vi "Washing Machine.vi"() -> ()   [LabVIEW 2026]
doc: "Timed cyclic state machine for a washing machine: Soak, Wash, Rinse, Spin."
panel:
  out "History":enum16{"Soak", "Wash", "Rinse", "Spin"}[](array[ring])
  out "Cycles":i32
  out "Final Tick":i32
  out "Final State":enum16{"Soak", "Wash", "Rinse", "Spin"}(ring)
  in  "Max Cycles":i32=2
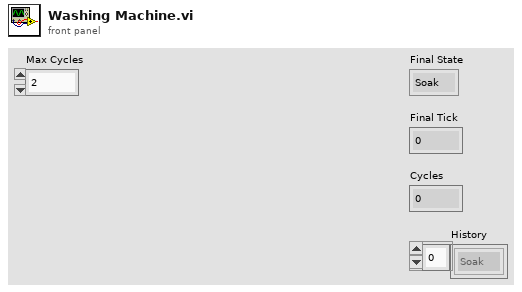
[diagram p1: front panel]
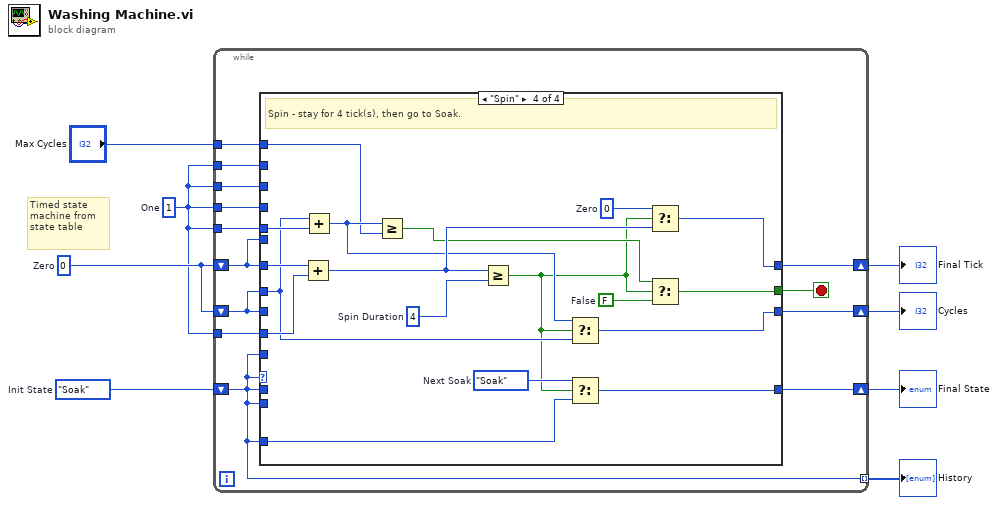
[diagram p0: block diagram]
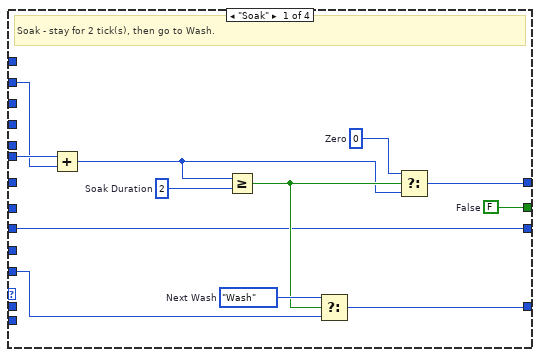
[diagram p2: hidden frame]
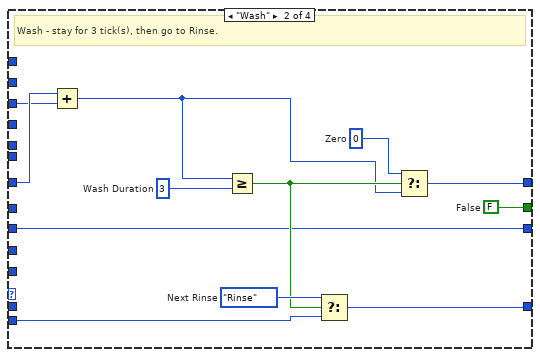
[diagram p3: hidden frame]
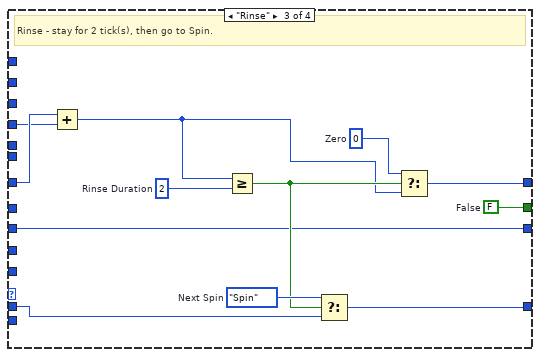
[diagram p4: hidden frame]
diagram:
  w5 = 1  # One
  w6 = 0  # Zero
  w7 = enum16{"Soak", "Wash", "Rinse", "Spin"}."Soak"  # Init State
  # "Timed state machine from state table"
  n1 = while {
    tunnel: "Max Cycles" -> [w14]
    tunnel: [w10] -> w1 mode=indexing
    shift-right: [w13] -> w4
    shift-left: w7 -> [w10]
    shift-right: [w12] -> w3
    shift-left: w6 -> [w18]
    shift-right: [w11] -> w2
    shift-left: w6 -> [w15]
    tunnel: w5 -> [w21]
    tunnel: w5 -> [w20]
    tunnel: w5 -> [w19]
    tunnel: w5 -> [w17]
    tunnel: w5 -> [w16]
    stop <- w9 stop-if-true
    n2 = case shown="\"Spin\"" w10 {
      tunnel: w18 -> [w33 _ _ _]
      tunnel: w21 -> [w32 _ _ _]
      tunnel: w10 -> [w29 _ _ _]
      tunnel: [w25 w37 w49 w61] -> w13
      tunnel: [w24 w36 w48 w60] -> w12
      tunnel: [w23 w35 w47 w59] -> w11
      tunnel: [w22 w34 w46 w58] -> w9
      tunnel: w20 -> [_ w44 _ _]
      tunnel: w10 -> [_ w41 _ _]
      tunnel: w19 -> [_ _ w56 _]
      tunnel: w10 -> [_ _ w53 _]
      tunnel: w15 -> [w23 w35 w47 _]
      tunnel: w18 -> [_ w45 w57 w75]
      tunnel: w17 -> [_ _ _ w74]
      tunnel: w10 -> [_ _ _ w71]
      tunnel: w16 -> [_ _ _ w68]
      tunnel: w15 -> [_ _ _ w67]
      tunnel: w14 -> [_ _ _ w65]
      frame "Soak" {
        w22 = FALSE  # False
        w28 = 0  # Zero
        w30 = enum16{"Soak", "Wash", "Rinse", "Spin"}."Wash"  # Next Wash
        w31 = 2  # Soak Duration
        # "Soak - stay for 2 tick(s), then go to Wash."
        n3 = Add(x=w33, y=w32) -> (x+y=w26:i32)
        n4 = Greater Or Equal?(x=w26, y=w31) -> (x >= y?=w27:bool)
        n5 = Select(t=w30, s=w27, f=w29) -> (s? t:f=w25:enum16{"Soak", "Wash", "Rinse", "Spin"})
        n6 = Select(t=w28, s=w27, f=w26) -> (s? t:f=w24:i32)
      }
      frame "Wash" {
        w34 = FALSE  # False
        w40 = 0  # Zero
        w42 = enum16{"Soak", "Wash", "Rinse", "Spin"}."Rinse"  # Next Rinse
        w43 = 3  # Wash Duration
        # "Wash - stay for 3 tick(s), then go to Rinse."
        n7 = Add(x=w45, y=w44) -> (x+y=w38:i32)
        n8 = Greater Or Equal?(x=w38, y=w43) -> (x >= y?=w39:bool)
        n9 = Select(t=w42, s=w39, f=w41) -> (s? t:f=w37:enum16{"Soak", "Wash", "Rinse", "Spin"})
        n10 = Select(t=w40, s=w39, f=w38) -> (s? t:f=w36:i32)
      }
      frame "Rinse" {
        w46 = FALSE  # False
        w52 = 0  # Zero
        w54 = enum16{"Soak", "Wash", "Rinse", "Spin"}."Spin"  # Next Spin
        w55 = 2  # Rinse Duration
        # "Rinse - stay for 2 tick(s), then go to Spin."
        n11 = Add(x=w57, y=w56) -> (x+y=w50:i32)
        n12 = Greater Or Equal?(x=w50, y=w55) -> (x >= y?=w51:bool)
        n13 = Select(t=w54, s=w51, f=w53) -> (s? t:f=w49:enum16{"Soak", "Wash", "Rinse", "Spin"})
        n14 = Select(t=w52, s=w51, f=w50) -> (s? t:f=w48:i32)
      }
      frame "Spin" {
        w62 = FALSE  # False
        w70 = 0  # Zero
        w72 = enum16{"Soak", "Wash", "Rinse", "Spin"}."Soak"  # Next Soak
        w73 = 4  # Spin Duration
        # "Spin - stay for 4 tick(s), then go to Soak."
        n15 = Add(x=w75, y=w74) -> (x+y=w69:i32)
        n16 = Add(x=w67, y=w68) -> (x+y=w66:i32)
        n17 = Greater Or Equal?(x=w66, y=w65) -> (x >= y?=w64:bool)
        n18 = Greater Or Equal?(x=w69, y=w73) -> (x >= y?=w63:bool)
        n19 = Select(t=w66, s=w63, f=w67) -> (s? t:f=w59:i32)
        n20 = Select(t=w72, s=w63, f=w71) -> (s? t:f=w61:enum16{"Soak", "Wash", "Rinse", "Spin"})
        n21 = Select(t=w70, s=w63, f=w69) -> (s? t:f=w60:i32)
        n22 = Select(t=w64, s=w63, f=w62) -> (s? t:f=w58:bool)
      }
    }
  }
  "Final State" <- w4
  "Final Tick" <- w3
  "Cycles" <- w2
  "History" <- w1
